vi "LB_ItemIndex_Tests.vi"(11 "error in":errorcluster) -> (15 "error out":errorcluster)   [LabVIEW 2016, in "DronaTest.lvlib"]
uses:
  DronaTest.lvlib
  APIs/Stimulus/ControlValue/SetValueAuto.vi
  APIs/Stimulus/ControlValue/Controls/Listbox/SetValueByItemIndex.vi
  APIs/Assert/AssertControlValue/Equal.vi
  APIs/Get/GetControlRef/GetControlRefByPath.vi
  <vilib>/addons/_JKI Toolkits/Caraya/classes/Test/Test.lvclass
  Drona.lvlib
  <vilib>/SLL Toolkit/SLL Debug/SLL Debug.lvlib
  APIs/Stimulus/ControlValue/Controls/Listbox/StimulusListbox.lvlib
  APIs/Assert/AssertControlValue/AssertControlValue.lvlib
  <vilib>/addons/_JKI Toolkits/Caraya/classes/Assert/Assert.lvclass
  APIs/Stimulus/ControlValue/ControlValue.lvlib
  APIs/Get/GetControlRef/GetControlRef.lvlib
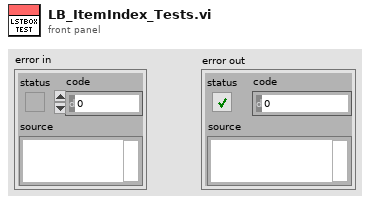
[diagram p1: front panel]
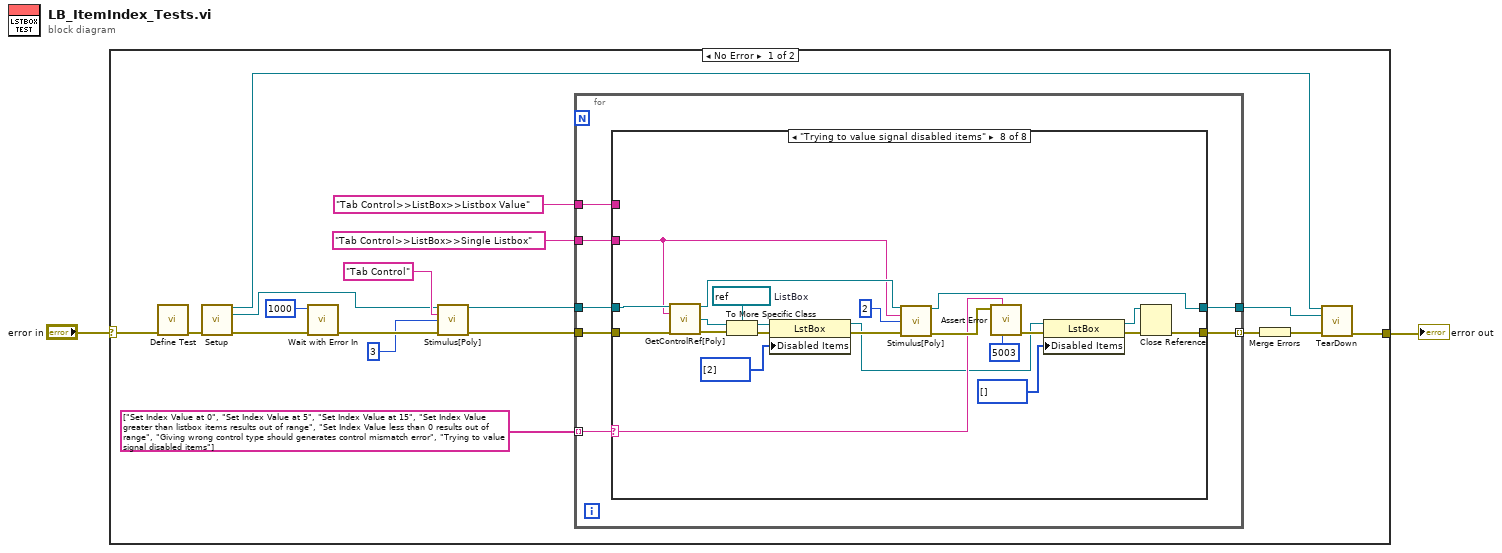
[diagram p0: block diagram]
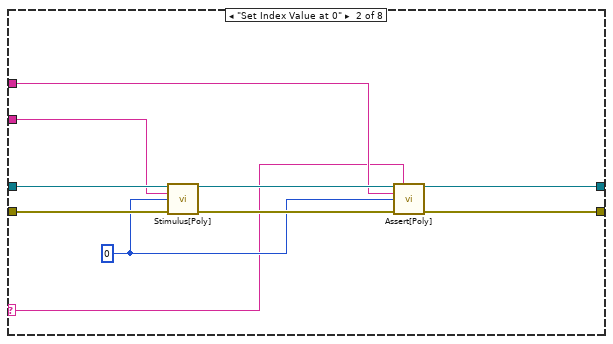
[diagram p3: hidden frame]
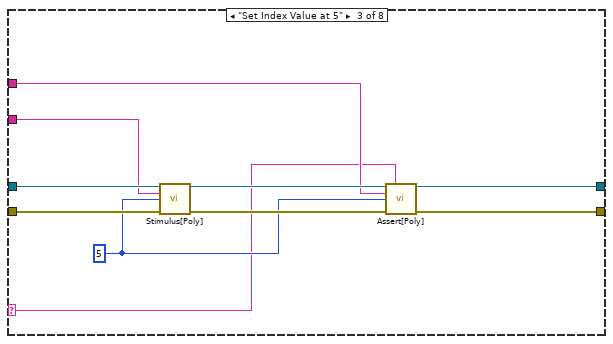
[diagram p4: hidden frame]
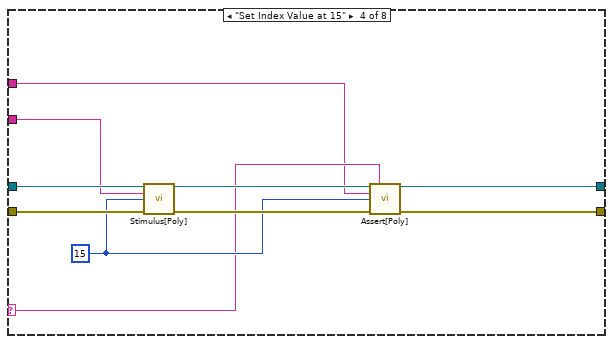
[diagram p5: hidden frame]
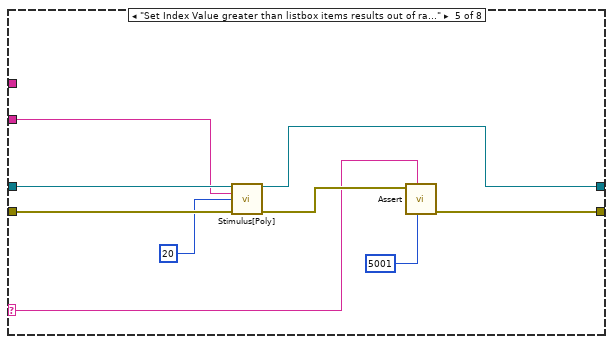
[diagram p6: hidden frame]
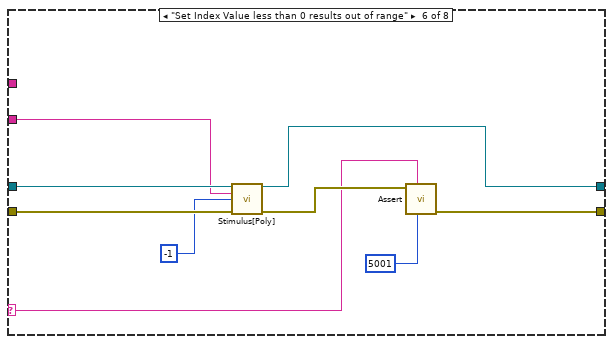
[diagram p7: hidden frame]
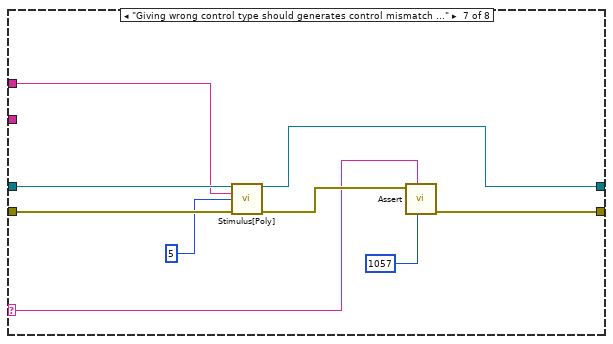
[diagram p8: hidden frame]
diagram:
  n1 = case shown="No Error" "error in" {
    selector: "error in" -> [w20 w109]
    tunnel: [w3 w109] -> w1
    frame No Error {
      n2 = call <vilib>:"Define Test.vi"("error in (no error)"=w20) -> ("error out"=w9:errorcluster)  [unwired: 9 in, 1 out]
      n3 = call "Setup.vi"("error in"=w9) -> ("Application Ref"=w5:refnum<vi>, "VI out"=w7:refnum<vi>, "error out"=w8:errorcluster)  [unwired: 12 in]
      n4 = call <vilib>:"Wait with Error In.vi"("error in (no error)"=w8, "milliseconds to wait"=u32 1000) -> ("error out"=w18:errorcluster)  [unwired: 9 in]
      n5 = call-poly "Stimulus[Poly].vi"("VI Reference In"=w7, "Control Path"="Tab Control", "Value (Signaling)"=3, "error in"=w18) -> ("VI Reference Out"=w14:refnum<vi>, "error out"=w17:errorcluster)  [unwired: 10 in]
      n6 = for {
        tunnel: w14 -> [w26]
        tunnel: "Tab Control>>ListBox>>Single Listbox" ("Control Path") -> [w25]
        tunnel: "Tab Control>>ListBox>>Listbox Value" ("Control Path") -> [w24]
        tunnel: string[] ["Set Index Value at 0", "Set Index Value at 5", "Set Index Value at 15", "Set Index Value greater than listbox items results out of range", "Set Index Value less than 0 results out of range", "Giving wrong control type should generates control mismatch error", "Trying to value signal disabled items"] -> [w22] mode=indexing
        tunnel: [w21] -> w4
        tunnel: w17 -> [w27]
        tunnel: [w23] -> w10 mode=indexing
        n7 = case shown="\"Trying to value signal disabled items\"" w22 {
          selector: w22 -> [_ w30 w40 w52 w62 w71 w81 w95]
          tunnel: w27 -> [w29 w39 w49 w59 w68 w77 w86 w103]
          tunnel: w26 -> [w28 w38 w48 w58 w67 w76 w85 w101]
          tunnel: w25 -> [_ w34 w44 w50 w65 w74 _ w87]
          tunnel: w24 -> [_ w33 w43 w51 _ _ w78 _]
          tunnel: [w29 w32 w42 w54 w63 w72 w82 w92] -> w23
          tunnel: [w28 w31 w41 w53 w60 w69 w79 w90] -> w21
          frame Default {
          }
          frame "Set Index Value at 0" {
            w35 = 0 ("Item Index")
            n8 = call-poly "Stimulus[Poly].vi"("VI Reference In"=w38, "Control Path"=w34, "Item Index"=w35, "Error In"=w39) -> ("VI Reference Out"=w36:refnum<vi>, "Error Out"=w37:errorcluster)  [unwired: 10 in]
            n9 = call-poly "Assert[Poly].vi"("VI Reference In"=w36, "Test Label"=w30, "Control Path"=w33, "Control Value"=w35, "Error In"=w37) -> ("VI Reference Out"=w31:refnum<vi>, "Error Out"=w32:errorcluster)  [unwired: 8 in, 1 out]
          }
          frame "Set Index Value at 5" {
            w45 = 5 ("Item Index")
            n10 = call-poly "Stimulus[Poly].vi"("VI Reference In"=w48, "Control Path"=w44, "Item Index"=w45, "Error In"=w49) -> ("VI Reference Out"=w46:refnum<vi>, "Error Out"=w47:errorcluster)  [unwired: 10 in]
            n11 = call-poly "Assert[Poly].vi"("VI Reference In"=w46, "Test Label"=w40, "Control Path"=w43, "Control Value"=w45, "Error In"=w47) -> ("VI Reference Out"=w41:refnum<vi>, "Error Out"=w42:errorcluster)  [unwired: 8 in, 1 out]
          }
          frame "Set Index Value at 15" {
            w55 = 15 ("Item Index")
            n12 = call-poly "Stimulus[Poly].vi"("VI Reference In"=w58, "Control Path"=w50, "Item Index"=w55, "Error In"=w59) -> ("VI Reference Out"=w56:refnum<vi>, "Error Out"=w57:errorcluster)  [unwired: 10 in]
            n13 = call-poly "Assert[Poly].vi"("VI Reference In"=w56, "Test Label"=w52, "Control Path"=w51, "Control Value"=w55, "Error In"=w57) -> ("VI Reference Out"=w53:refnum<vi>, "Error Out"=w54:errorcluster)  [unwired: 8 in, 1 out]
          }
          frame "Set Index Value greater than listbox items results out of range" {
            n14 = call-poly "Stimulus[Poly].vi"("VI Reference In"=w67, "Control Path"=w65, "Item Index"=20, "Error In"=w68) -> ("VI Reference Out"=w60:refnum<vi>, "Error Out"=w64:errorcluster)  [unwired: 10 in]
            n15 = call-poly <vilib>:"Assert.vi"("error code (1)"=5001, "Label"=w62, "Error?"=w64) -> ("error out"=w63:errorcluster)  [unwired: 7 in, 1 out]
          }
          frame "Set Index Value less than 0 results out of range" {
            n16 = call-poly "Stimulus[Poly].vi"("VI Reference In"=w76, "Control Path"=w74, "Item Index"=-1, "Error In"=w77) -> ("VI Reference Out"=w69:refnum<vi>, "Error Out"=w73:errorcluster)  [unwired: 10 in]
            n17 = call-poly <vilib>:"Assert.vi"("error code (1)"=5001, "Label"=w71, "Error?"=w73) -> ("error out"=w72:errorcluster)  [unwired: 7 in, 1 out]
          }
          frame "Giving wrong control type should generates control mismatch error" {
            n18 = call-poly "Stimulus[Poly].vi"("VI Reference In"=w85, "Control Path"=w78, "Item Index"=5, "Error In"=w86) -> ("VI Reference Out"=w79:refnum<vi>, "Error Out"=w83:errorcluster)  [unwired: 10 in]
            n19 = call-poly <vilib>:"Assert.vi"("error code (1)"=1057, "Label"=w81, "Error?"=w83) -> ("error out"=w82:errorcluster)  [unwired: 7 in, 1 out]
          }
          frame "Trying to value signal disabled items" {
            w107 = refnum<vi> refnum  # ListBox
            n20 = call-poly "GetControlRef[Poly].vi"("VI Reference In"=w101, "Control Path"=w87, "error In"=w103) -> ("VI Reference Out"=w100:refnum<vi>, "Ctl Refnum"=w99:refnum<vi>, "error out"=w102:errorcluster)  [unwired: 10 in]
            n21 = To More Specific Class(target class=w107, reference=w99, error in=w102) -> (specific class reference=w106:refnum<vi>, error out=w108:errorcluster)
            n22 = property class="LstBox"(reference=w106, error in=w108, "Disabled Items"=i32[] [2]) -> (reference out=w89:refnum<vi>, error out=w104:errorcluster)
            n23 = call-poly "Stimulus[Poly].vi"("VI Reference In"=w100, "Control Path"=w87, "Item Index"=2, "Error In"=w104) -> ("VI Reference Out"=w90:refnum<vi>, "Error Out"=w96:errorcluster)  [unwired: 10 in]
            n24 = call <vilib>:"Assert Error.vi"("error code (1)"=5003, "Label"=w95, "Error?"=w96) -> ("error out"=w94:errorcluster)  [unwired: 7 in, 1 out]
            n25 = property class="LstBox"(reference=w89, error in=w94, "Disabled Items"=i32[] []) -> (reference out=w91:refnum<vi>, error out=w93:errorcluster)
            n26 = Close Reference(reference=w91, error in (no error)=w93) -> (error out=w92:errorcluster)
          }
        }
      }
      n27 = Merge Errors(w10) -> (w6:errorcluster)
      n28 = call "TearDown.vi"("Application Ref"=w5, "VI in"=w4, "error in (no error)"=w6) -> ("error out"=w3:errorcluster)  [unwired: 12 in]
    }
    frame Error {
    }
  }
  "error out" <- w1
